vi "数据分类.vi"(5 "包含删除？":T1, 6 "所有类型":bool, 7 "测试类型":T2, 11 "数组输入":T3[](array[typedef])) -> (1 "数据索引":i32[](array[numeric]), 3 "数组输出":T3[](array[typedef]))   [LabVIEW 2020]
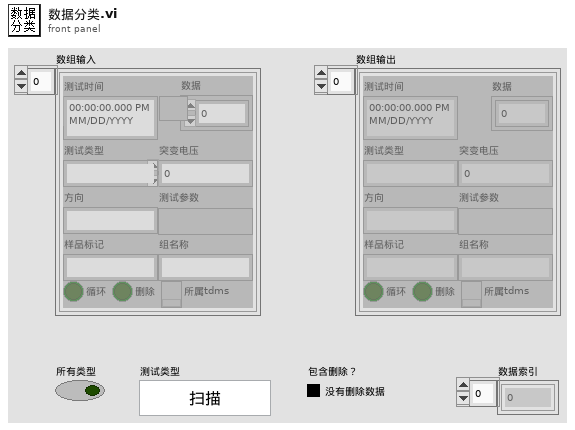
[diagram p1: front panel]
types:
  T1 = typedef "包含删除.ctl" = enum8{"False", "True", "Mixed"}
  T2 = typedef "测试类型.ctl" = enum16{"扫描", "保持时间", "脉冲", "高速脉冲", "任意波形"}
  T3 = typedef "测试数据类型.ctl" = cluster{"测试时间":timestamp, "数据":dbl[][], "测试类型":string, "方向":string, "样品标记":string, "突变电压":i32, "测试参数":variant, "循环":bool, "删除":bool, "组名称":string, "所属tdms":refnum<k34>}
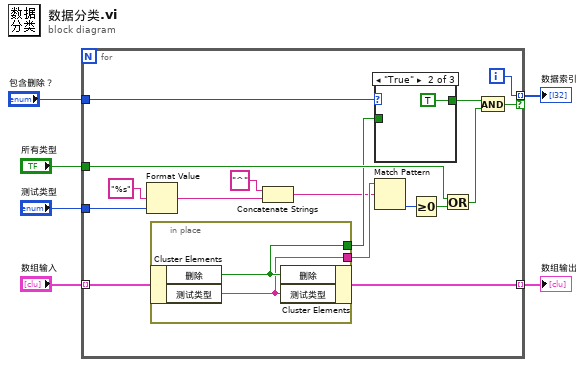
[diagram p0: block diagram]
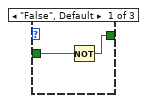
[diagram p2: hidden frame]
diagram:
  n1 = for {
    tunnel: "数组输入" -> [w23] mode=indexing
    tunnel: [w22] -> w6 mode=indexing
    tunnel: "测试类型" -> [w16]
    tunnel: "所有类型" -> [w21]
    tunnel: "包含删除？" -> [w20]
    tunnel: [w15] -> w1 mode=indexing if=w14
    i -> [w15]
    n2 = Format Value(format string="%s" ("格式字符串"), value (0)=w16) -> (output string=w11:string)  [unwired: 1 in]
    n3 = in-place {
      in-place-border: [w29] -> w19
      in-place-border: [w28] -> w12
      n4 = in-place-cluster #1(w23) -> ("删除"=w29:bool, "测试类型"=w28:string)
      n5 = in-place-cluster #1("删除"=w29, "测试类型"=w28) -> (w22:T3)
    }
    n6 = Concatenate Strings("^" ("字符串"), w11) -> (w8:string)
    n7 = case shown="\"True\"" w20 {
      tunnel: w19 -> [w25 _ w27]
      tunnel: [w24 TRUE w27] -> w17
      frame "False", Default {
        n8 = Not(x=w25) -> (.not. x?=w24:bool)
      }
      frame "True" {
      }
      frame "Mixed" {
      }
    }
    n9 = Match Pattern(string=w12, regular expression=w8) -> (offset past match=w10:i32)  [unwired: 1 in, 3 out]
    n10 = Greater Or Equal To 0?(x=w10) -> (x >= 0?=w9:bool)
    n11 = Or(x=w21, y=w9) -> (x .or. y?=w18:bool)
    n12 = And(x=w17, y=w18) -> (x .and. y?=w14:bool)
  }
  "数组输出" <- w6
  "数据索引" <- w1
